vi "Image Generator.vi"(4 "Coerce":bool, 6 "Hide Labels":bool, 7 "Lithography Data":T2(array[cluster]), 8 "error in (no error)":errorcluster, 9 "Resolution":i32=444, 11 "Image Reference In":T3) -> (0 "error out":errorcluster, 3 "Image Reference Out":T3)   [LabVIEW 2019]
doc: "This VI generates a rendered image given the lithography data."
uses:
  <vilib>/vision/Image Controls.llb/IMAQ Image.ctl
  <userlib>/LevyLab/Relay Box/Typedefs/Resistor--enum.ctl
  Global Variables.vi
  <userlib>/LevyLab/Relay Box/Relay-Box.lvclass
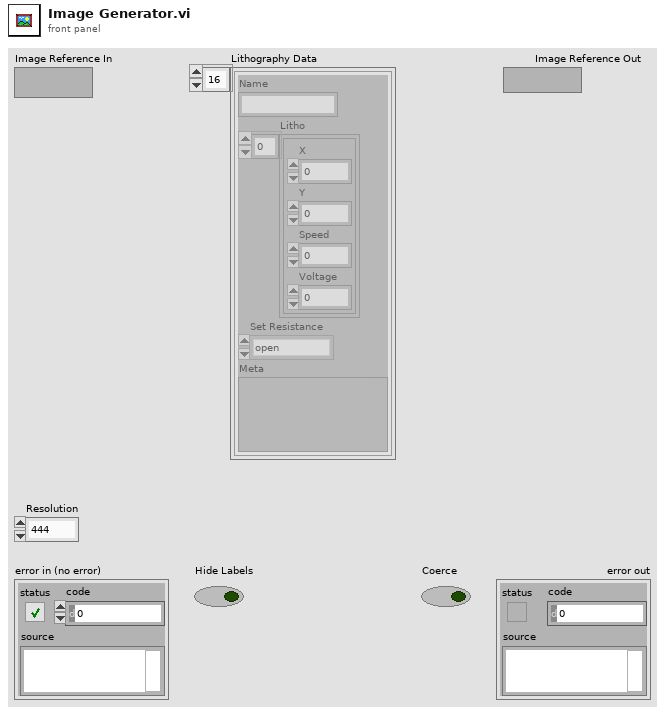
[diagram p1: front panel]
types:
  T1 = typedef "Relay-Box.lvclass/Resistor--enum.ctl" = enum16{"open", "discharge tip", "0 ohms", "100k ohm", "10M ohm", "1G ohm"}
  T2 = cluster{"Name":string, "Litho":cluster{"X":dbl, "Y":dbl, "Speed":dbl, "Voltage":dbl}[], "Set Resistance":T1, "Meta":variant}[]
  T3 = typedef "IMAQ Image.ctl" = refnum<image>
  T4 = cluster{"X":dbl, "Y":dbl, "Speed":dbl, "Voltage":dbl}
  T5 = cluster{"X":dbl, "Y":dbl, "Speed":dbl, "Voltage":dbl}[]
  T6 = cluster{"X":bool, "Y":bool, "Speed":bool, "Voltage":bool}
  T7 = cluster{"Name":string, "Litho":cluster{"X":dbl, "Y":dbl, "Speed":dbl, "Voltage":dbl}[], "Set Resistance":T1, "Meta":variant}
  T8 = cluster{"Desired Font (Application)":enum16{"User-specified Font", "Application Font", "System Font", "Dialog Font"}, "[User-specified Font]":cluster{"Font Name":string, "Size":i16, "Strikeout?":bool, "Italic?":bool, "Underline?":bool, "Outline?":bool, "Shadow?":bool, "Bold?":bool, "Rotation Angle":dbl}, "Horizontal Alignment":i16, "Vertical Alignment":i16}
  T9 = cluster{"Left":i32, "Top":i32, "Right":i32, "Bottom":i32}
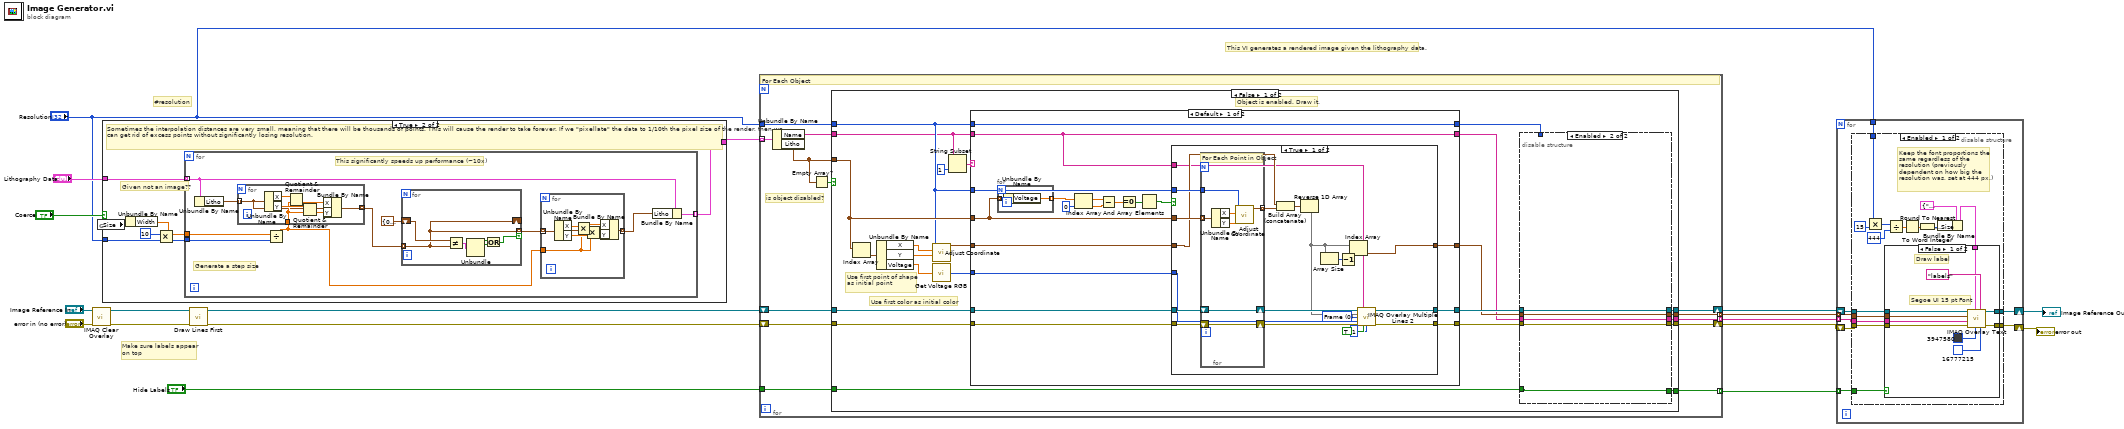
[diagram p0: block diagram]
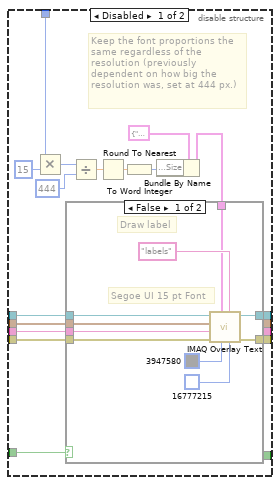
[diagram p5: hidden frame]
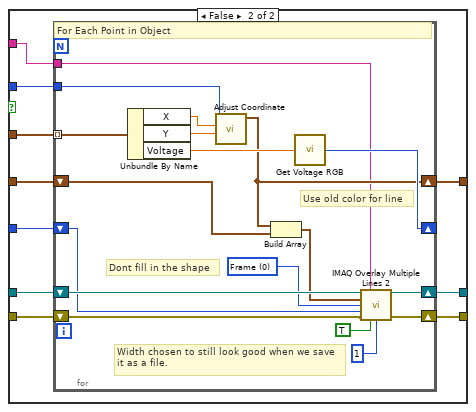
[diagram p7: hidden frame]
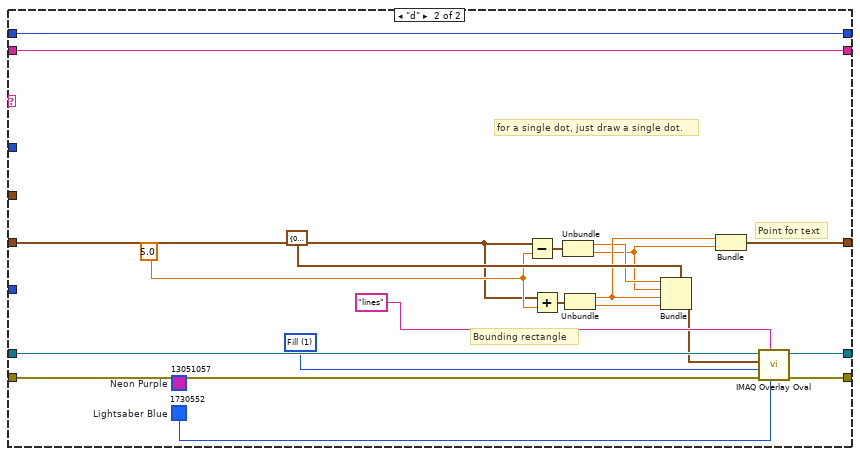
[diagram p8: hidden frame]
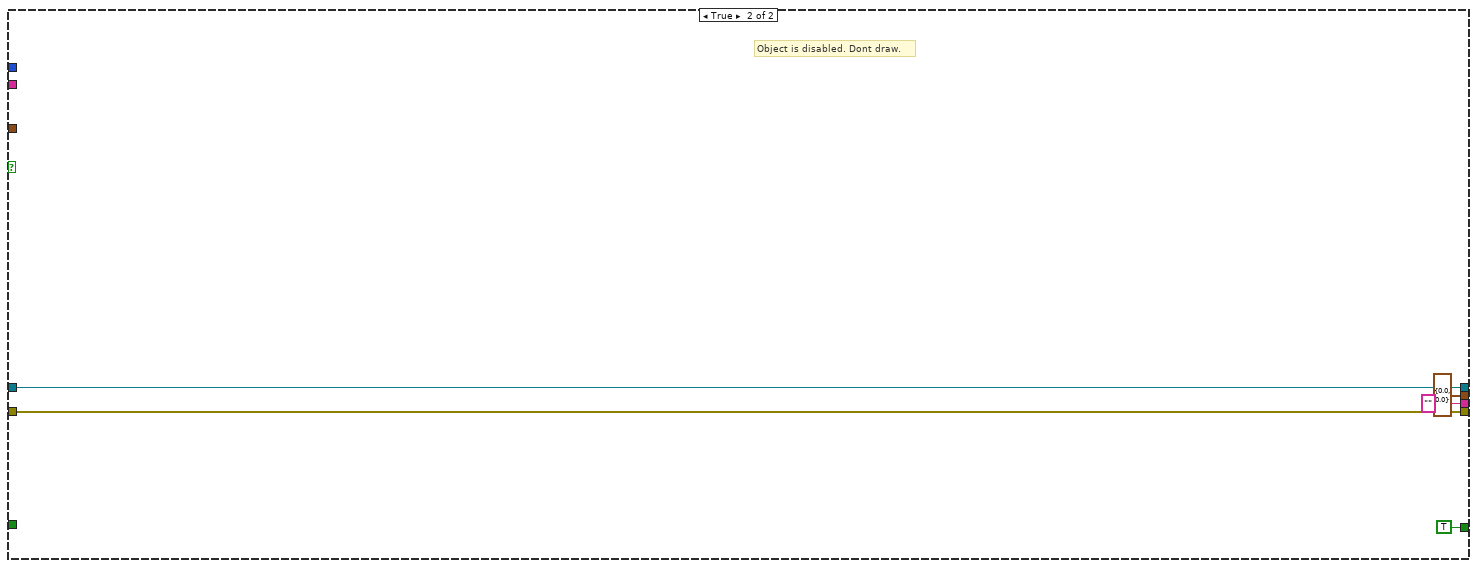
[diagram p9: hidden frame]
diagram:
  # "Make sure labels appear\non top"
  # "#resolution"
  # "This VI generates a rendered image given the lithography data."
  n1 = call "IMAQ Clear Overlay"("Image"="Image Reference In") -> ("Image Out"=w2:T3)  [unwired: 9 in, 1 out]
  n2 = case shown="True" "Coerce" {
    tunnel: "Lithography Data" -> [w18 w21]
    tunnel: [w18 w20] -> w4
    tunnel: "Resolution" -> [_ w19]
    frame False {
    }
    frame True {
      # "Given not an image??"
      # "Sometimes the interpolation distances are very small, meaning that there will be thousands of points. This will cause the render to take forever. If we \"pixellate\" the data to 1/10th the pixel size of the render, then we can get rid of excess points without significantly losing resolution."
      n3 = global read "Global Variables.vi" "Size"() -> (w25:cluster{"Width":dbl, "Height":dbl})
      n4 = Unbundle By Name(w25) -> ("Width"=w24:dbl)
      n5 = Multiply(x=10, y=w19) -> (x*y=w23:i32)
      n6 = for {
        tunnel: w24 -> [w35]
        tunnel: w23 -> [w33]
        tunnel: w21 -> [w30] mode=indexing
        tunnel: [w29] -> w20 mode=indexing
        # "This significantly speeds up performance (~10x)"
        # "Generate a step size"
        n7 = Unbundle By Name(w30) -> ("Litho"=w34:T5)
        n8 = Divide(x=w35, y=w33) -> (x/y=w26:dbl)
        n9 = for {
          tunnel: w34 -> [w43] mode=indexing
          tunnel: [w44] -> w31 mode=indexing
          tunnel: w26 -> [w47]
          n10 = Unbundle By Name(w43) -> ("X"=w49:dbl, "Y"=w48:dbl)
          n11 = Quotient & Remainder(x=w49, y=w47) -> (floor(x/y)=w46:dbl)  [unwired: 1 out]
          n12 = Quotient & Remainder(x=w48, y=w47) -> (floor(x/y)=w45:dbl)  [unwired: 1 out]
          n13 = Bundle By Name(cluster=w43, "X"=w46, "Y"=w45) -> (w44:T4)
        }
        n14 = for {
          shift-right: [w50] -> _
          shift-left: T4 {"X"=0.0, "Y"=0.0, "Speed"=0.0, "Voltage"=0.0} ("Litho Point") -> [w55]
          tunnel: [w50] -> w27 mode=indexing if=w51
          tunnel: w31 -> [w50] mode=indexing
          n15 = Not Equal?(x=w55, y=w50) -> (x != y?=w54:T6)
          n16 = Unbundle(w54) -> ("X"=w53:bool, "Y"=w52:bool)  [unwired: 2 out]
          n17 = Or(x=w53, y=w52) -> (x .or. y?=w51:bool)
        }
        n18 = for {
          tunnel: [w39] -> w28 mode=indexing
          tunnel: w27 -> [w40] mode=indexing
          tunnel: w26 -> [w36]
          n19 = Unbundle By Name(w40) -> ("X"=w42:dbl, "Y"=w41:dbl)
          n20 = Multiply(x=w42, y=w36) -> (x*y=w38:dbl)
          n21 = Multiply(x=w36, y=w41) -> (x*y=w37:dbl)
          n22 = Bundle By Name(cluster=w40, "X"=w38, "Y"=w37) -> (w39:T4)
        }
        n23 = Bundle By Name(cluster=w30, "Litho"=w28) -> (w29:T7)
      }
    }
  }
  n24 = call "Draw Lines First.vi"("error in (no error)"="error in (no error)", "Refnum in"=w2) -> ("error out"=w16:errorcluster, "Refnum out"=w17:T3)  [unwired: 8 in]
  n25 = for {
    tunnel: w4 -> [w66] mode=indexing
    shift-right: [w67] -> w10
    shift-left: w16 -> [w68]
    tunnel: "Resolution" -> [w64]
    tunnel: "Hide Labels" -> [w60]
    shift-right: [w59] -> w11
    shift-left: w17 -> [w65]
    tunnel: [w58] -> w14 mode=indexing
    tunnel: [w57] -> w13 mode=indexing
    tunnel: [w56] -> w12 mode=indexing
    # "is object disabled?"
    # "For Each Object"
    n26 = Unbundle By Name(w66) -> ("Name"=w63:string, "Litho"=w61:T5)
    n27 = Empty Array?(array=w61) -> (empty?=w62:bool)
    n28 = case shown="False" w62 {
      tunnel: w68 -> [w92 w223]
      tunnel: [w90 w223] -> w67
      tunnel: [w88 w224] -> w59
      tunnel: w61 -> [w87 _]
      tunnel: w65 -> [w79 w224]
      tunnel: w64 -> [w78 _]
      tunnel: w63 -> [w75 _]
      tunnel: w60 -> [w72 _]
      tunnel: [w71 cluster{dbl, dbl} {0.0, 0.0} ("Adjusted Coordinate")] -> w58
      tunnel: [w70 "" ("Name")] -> w57
      tunnel: [w69 TRUE ("Hide Labels")] -> w56
      frame False {
        # "Object is enabled. Draw it."
        # "Use first color as initial color"
        # "Use first point of shape as initial point"
        n29 = Index Array(array=w87) -> (element=w86:T4)  [unwired: 1 in]
        n30 = Unbundle By Name(w86) -> ("X"=w84:dbl, "Y"=w83:dbl, "Voltage"=w85:dbl)
        n31 = call "Adjust Coordinate.vi"("Y"=w83, "X"=w84, "Resolution"=w78) -> ("Adjusted Coordinate"=w81:cluster{dbl, dbl})  [unwired: 7 in, 1 out]
        n32 = call "Get Voltage RGB.vi"("Voltage"=w85) -> ("RGB Value"=w82:u32)  [unwired: 3 in, 1 out]
        n33 = String Subset(string=w75, length (rest)=1 ("length (rest)")) -> (substring=w73:string)  [unwired: 1 in]
        n34 = case shown="Default" w73 {
          tunnel: w92 -> [w142 w203]
          tunnel: [w141 w217] -> w91
          tunnel: [w140 w216] -> w89
          tunnel: w87 -> [w133 _]
          tunnel: w82 -> [w139 _]
          tunnel: w81 -> [w138 w201]
          tunnel: [w137 w200] -> w80
          tunnel: w79 -> [w136 w215]
          tunnel: w78 -> [w135 _]
          tunnel: w75 -> [w126 w218]
          tunnel: w78 -> [w134 w219]
          tunnel: [w126 w218] -> w77
          tunnel: [w134 w219] -> w76
          frame Default {
            n35 = for {
              tunnel: w133 -> [w199] mode=indexing
              tunnel: [w198] -> w131 mode=indexing
              n36 = Unbundle By Name(w199) -> ("Voltage"=w198:dbl)
            }
            n37 = Index Array(array=w131, index=0) -> (element=w130:dbl)
            n38 = Subtract(x=w131, y=w130) -> (x-y=w129:dbl[])
            n39 = Equal To 0?(x=w129) -> (x = 0?=w128:bool[])
            n40 = And Array Elements(Boolean array=w128) -> (logical AND=w127:bool)
            n41 = case shown="True" w127 {
              tunnel: w142 -> [w162 w179]
              tunnel: [w157 w178] -> w141
              tunnel: [w155 w177] -> w140
              tunnel: w139 -> [w153 w176]
              tunnel: w138 -> [w147 w175]
              tunnel: [w148 w171] -> w137
              tunnel: w136 -> [w161 w174]
              tunnel: w135 -> [w160 w173]
              tunnel: w133 -> [w159 w172]
              tunnel: w126 -> [w143 w170]
              frame True {
                w154 = u32 0 items=["Frame", "Fill"] ("Drawing Mode (Frame)")
                n42 = for {
                  tunnel: w159 -> [w169] mode=indexing
                  shift-right: [w165] -> w156
                  shift-left: w161 -> [w165]
                  shift-right: [w164] -> w158
                  shift-left: w162 -> [w164]
                  tunnel: w160 -> [w166]
                  tunnel: [w163] -> w145 mode=indexing
                  # "For Each Point in Object"
                  n43 = Unbundle By Name(w169) -> ("X"=w168:dbl, "Y"=w167:dbl)
                  n44 = call "Adjust Coordinate.vi"("Y"=w167, "X"=w168, "Resolution"=w166) -> ("Adjusted Coordinate"=w163:cluster{dbl, dbl})  [unwired: 7 in, 1 out]
                }
                n45 = Build Array (concatenate)(w147, w145) -> (w146:cluster{dbl, dbl}[])
                n46 = Reverse 1D Array(array=w146) -> (reversed array=w144:cluster{dbl, dbl}[])
                n47 = Array Size(array=w144) -> (size(s)=w150:i32)
                n48 = Decrement(x=w150) -> (x-1=w149:i32)
                n49 = Index Array(array=w144, index=w149) -> (element=w148:cluster{dbl, dbl})
                n50 = call "IMAQ Overlay Multiple Lines 2"("Image"=w156, "Group"=w143, "Line End Points"=w144, "Drawing Mode (Frame)"=w154, "Color"=w153, "error in (no error)"=w158, "Maintain Width?"=TRUE, "Width"=u32 1) -> ("Image Out"=w155:T3, "error out"=w157:errorcluster)  [unwired: 6 in]
              }
              frame False {
                n51 = for {
                  tunnel: w172 -> [w195] mode=indexing
                  shift-right: [w197] -> w177
                  shift-left: w174 -> [w191]
                  shift-right: [w196] -> w178
                  shift-left: w179 -> [w187]
                  shift-right: [w190] -> _
                  shift-left: w176 -> [w183]
                  shift-right: [w185] -> w171
                  shift-left: w175 -> [w186]
                  tunnel: w173 -> [w189]
                  tunnel: w170 -> [w180]
                  w181 = u32 0 items=["Frame", "Fill"] ("Drawing Mode (Frame)")
                  # "Dont fill in the shape"
                  # "Width chosen to still look good when we save it as a file."
                  # "Use old color for line"
                  # "For Each Point in Object"
                  n52 = Unbundle By Name(w195) -> ("X"=w193:dbl, "Y"=w192:dbl, "Voltage"=w194:dbl)
                  n53 = call "Adjust Coordinate.vi"("Y"=w192, "X"=w193, "Resolution"=w189) -> ("Adjusted Coordinate"=w185:cluster{dbl, dbl})  [unwired: 7 in, 1 out]
                  n54 = Build Array(w185, w186) -> (w184:cluster{dbl, dbl}[])
                  n55 = call "Get Voltage RGB.vi"("Voltage"=w194) -> ("RGB Value"=w190:u32)  [unwired: 3 in, 1 out]
                  n56 = call "IMAQ Overlay Multiple Lines 2"("Image"=w191, "Group"=w180, "Line End Points"=w184, "Drawing Mode (Frame)"=w181, "Color"=w183, "error in (no error)"=w187, "Maintain Width?"=TRUE, "Width"=u32 1) -> ("Image Out"=w197:T3, "error out"=w196:errorcluster)  [unwired: 6 in]
                }
              }
            }
          }
          frame "d" {
            w202 = u32 1730552  # Lightsaber Blue
            (unwired) u32 13051057  # Neon Purple
            w209 = u32 1 items=["Frame", "Fill"] ("Drawing Mode (Frame)")
            w207 = 5.0
            # "Point for text"
            # "Bounding rectangle"
            # "for a single dot, just draw a single dot."
            n57 = Subtract(x=w201, y=w207) -> (x-y=w212:cluster{dbl, dbl})
            n58 = Add(x=w201, y=w207) -> (x+y=w210:cluster{dbl, dbl})
            n59 = Unbundle(w212) -> (w205:dbl, w204:dbl)
            n60 = Unbundle(w210) -> (w206:dbl, w208:dbl)
            n61 = Bundle(cluster=T9 {"Left"=0, "Top"=0, "Right"=0, "Bottom"=0} ("Bounding Rectangle"), "Left"=w205, "Top"=w204, "Right"=w206, "Bottom"=w208) -> (w211:T9)
            n62 = Bundle(w206, w204) -> (w200:cluster{dbl, dbl})  [unwired: 1 in]
            n63 = call "IMAQ Overlay Oval"("Color"=w202, "Group"="lines", "error in (no error)"=w203, "Drawing Mode (Frame)"=w209, "Bounding Rectangle"=w211, "Image"=w215) -> ("error out"=w217:errorcluster, "Image Out"=w216:T3)  [unwired: 4 in]
          }
        }
        n64 = disable-structure shown="Enabled" {
          disable-tunnel: w91 -> [w108 w124]
          disable-tunnel: [w107 w124] -> w90
          disable-tunnel: w89 -> [w106 w125]
          disable-tunnel: [w105 w125] -> w88
          disable-tunnel: w80 -> [w104 w123]
          disable-tunnel: w77 -> [w95 w122]
          disable-tunnel: w76 -> [w94 _]
          disable-tunnel: w72 -> [w93 w121]
          disable-tunnel: [_ w123] -> w71
          disable-tunnel: [_ w122] -> w70
          disable-tunnel: [_ w121] -> w69
          frame Disabled {
            # "Keep the font proportions the same regardless of the resolution (previously dependent on how big the resolution was, set at 444 px.)"
            n65 = Multiply(x=w94, y=15) -> (x*y=w100:i32)
            n66 = Divide(x=w100, y=444) -> (x/y=w98:dbl)
            n67 = Round To Nearest(number=w98) -> (nearest integer value=w97:dbl)
            n68 = To Word Integer(number=w97) -> (16bit integer=w96:i16)
            n69 = Bundle By Name(cluster=T8 {"Desired Font (Application)"=enum."User-specified Font", "[User-specified Font]"={"Font Name"="Segoe UI", "Size"=35, "Strikeout?"=FALSE, "Italic?"=FALSE, "Underline?"=FALSE, "Outline?"=FALSE, "Shadow?"=FALSE, "Bold?"=FALSE, "Rotation Angle"=0.0}, "Horizontal Alignment"=0, "Vertical Alignment"=0} ("Font, Size & Style"), "[User-specified Font].Size"=w96) -> (w102:T8)
            n70 = case shown="False" w93 {
              tunnel: w108 -> [w118 w120]
              tunnel: [w117 w120] -> w107
              tunnel: w106 -> [w116 w119]
              tunnel: [w115 w119] -> w105
              tunnel: w104 -> [w109 _]
              tunnel: w102 -> [w111 _]
              tunnel: w95 -> [w110 _]
              frame False {
                # "Segoe UI 15 pt Font"
                # "Draw label"
                n71 = call "IMAQ Overlay Text"("BG Color (Transparent)"=u32 16777215, "Group"="labels", "Text Color (black)"=u32 3947580, "Font, Size & Style"=w111, "error in (no error)"=w118, "String"=w110, "Origin"=w109, "Image"=w116) -> ("error out"=w117:errorcluster, "Image Out"=w115:T3)  [unwired: 2 in]
              }
              frame True {
              }
            }
          }
          frame Enabled {
          }
        }
      }
      frame True {
        # "Object is disabled. Dont draw."
      }
    }
  }
  n72 = for {
    shift-right: [w232] -> w9
    shift-left: w11 -> [w229]
    shift-right: [w231] -> w8
    shift-left: w10 -> [w230]
    tunnel: w14 -> [w228] mode=indexing
    tunnel: w13 -> [w227] mode=indexing
    tunnel: w12 -> [w226] mode=indexing
    tunnel: "Resolution" -> [w225]
    n73 = disable-structure shown="Enabled" {
      disable-tunnel: w230 -> [w248 w261]
      disable-tunnel: [w247 w261] -> w231
      disable-tunnel: w229 -> [w246 w262]
      disable-tunnel: [w245 w262] -> w232
      disable-tunnel: w228 -> [w244 _]
      disable-tunnel: w227 -> [w235 _]
      disable-tunnel: w225 -> [w234 _]
      disable-tunnel: w226 -> [w233 _]
      frame Enabled {
        # "Keep the font proportions the same regardless of the resolution (previously dependent on how big the resolution was, set at 444 px.)"
        n74 = Multiply(x=w234, y=15) -> (x*y=w240:i32)
        n75 = Divide(x=w240, y=444) -> (x/y=w238:dbl)
        n76 = Round To Nearest(number=w238) -> (nearest integer value=w237:dbl)
        n77 = To Word Integer(number=w237) -> (16bit integer=w236:i16)
        n78 = Bundle By Name(cluster=T8 {"Desired Font (Application)"=enum."User-specified Font", "[User-specified Font]"={"Font Name"="Segoe UI", "Size"=35, "Strikeout?"=FALSE, "Italic?"=FALSE, "Underline?"=FALSE, "Outline?"=FALSE, "Shadow?"=FALSE, "Bold?"=FALSE, "Rotation Angle"=0.0}, "Horizontal Alignment"=0, "Vertical Alignment"=0} ("Font, Size & Style"), "[User-specified Font].Size"=w236) -> (w242:T8)
        n79 = case shown="False" w233 {
          tunnel: w248 -> [w258 w260]
          tunnel: [w257 w260] -> w247
          tunnel: w246 -> [w256 w259]
          tunnel: [w255 w259] -> w245
          tunnel: w244 -> [w249 _]
          tunnel: w242 -> [w251 _]
          tunnel: w235 -> [w250 _]
          frame False {
            # "Segoe UI 15 pt Font"
            # "Draw label"
            n80 = call "IMAQ Overlay Text"("BG Color (Transparent)"=u32 16777215, "Group"="labels", "Text Color (black)"=u32 3947580, "Font, Size & Style"=w251, "error in (no error)"=w258, "String"=w250, "Origin"=w249, "Image"=w256) -> ("error out"=w257:errorcluster, "Image Out"=w255:T3)  [unwired: 2 in]
          }
          frame True {
          }
        }
      }
      frame Disabled {
      }
    }
  }
  "Image Reference Out" <- w9
  "error out" <- w8
